vi "write commands.vi"(8 "error in":errorcluster, 9 "Timeout (ms)":i32=-1, 10 "commands":T1[](array[typedef]), 11 "profibus reference":T3) -> (0 "error out":errorcluster, 1 "Empty Elements Remaining":u32, 3 "profibus reference out":T3)   [LabVIEW 2013, in "dynamic profibus.lvlib"]
uses:
  dynamic profibus.lvlib
  fpga reference.ctl
  full command.ctl
  profibus master action.ctl
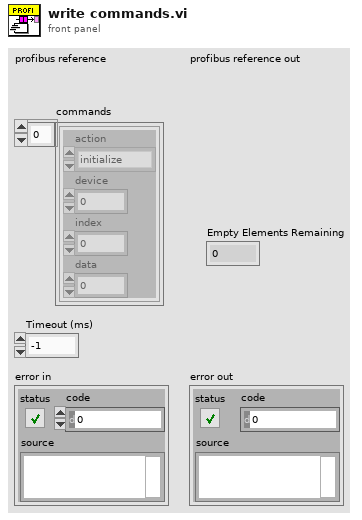
[diagram p1: front panel]
types:
  T1 = typedef "dynamic profibus.lvlib/full command.ctl" = cluster{"action":T2, "device":u8, "index":u8, "data":u8}
  T2 = typedef "dynamic profibus.lvlib/profibus master action.ctl" = enum8{"initialize", "uninitialize", "stop", "get input", "get input size", "set output", "get output size", "get diagnostic", "transfer data", "transfer diagnostics", "read many inputs"}
  T3 = typedef "dynamic profibus.lvlib/fpga reference.ctl" = refnum<k20>
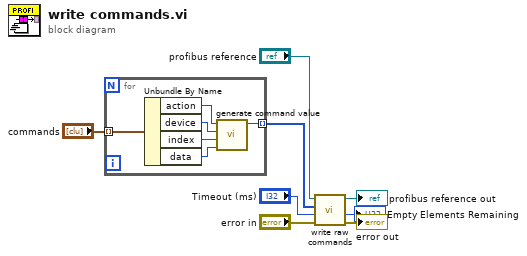
[diagram p0: block diagram]
diagram:
  n1 = for {
    tunnel: [w14] -> w3 mode=indexing
    tunnel: "commands" -> [w13] mode=indexing
    n2 = Unbundle By Name(w13) -> ("action"=w9:T2, "device"=w10:u8, "index"=w12:u8, "data"=w11:u8)
    n3 = call "generate command value.vi"("data"=w11, "index"=w12, "device"=w10, "action"=w9) -> ("Element"=w14:u32)  [unwired: 7 in]
  }
  n4 = call "write raw commands.vi"("error in"="error in", "Timeout (ms)"="Timeout (ms)", "Data"=w3, "profibus reference"="profibus reference") -> ("error out"=→"error out":errorcluster, "Empty Elements Remaining"=→"Empty Elements Remaining":u32, "profibus reference out"=→"profibus reference out":T3)  [unwired: 5 in]
